vi "Utility - Set 32x32 Picture Values.vi"(8 "error in":errorcluster, 10 "Icon Names":string, 11 "Picture Refnums":refnum<vi>[](array[refnum])) -> (0 "error out":errorcluster)   [LabVIEW 2014]
doc: "::: VI Helpeks :::\nCopyright (c) 2000-2026 Konstantin Shifershteyn. All rights reserved."
panel:
  # "VI Helpeks\nCopyright (c) 2012-2026 Konstantin Shifershteyn"
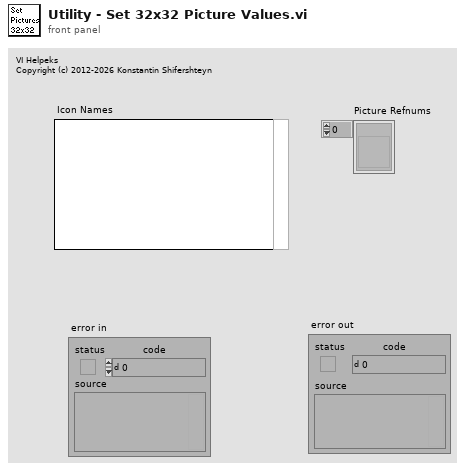
[diagram p1: front panel]
types:
  T1 = typedef "imagedata.ctl" = cluster{"image type":i32, "image depth":i32, "image":u8[], "mask":u8[], "colors":u32[], "Rectangle":cluster{"left":i16, "top":i16, "right":i16, "bottom":i16}}
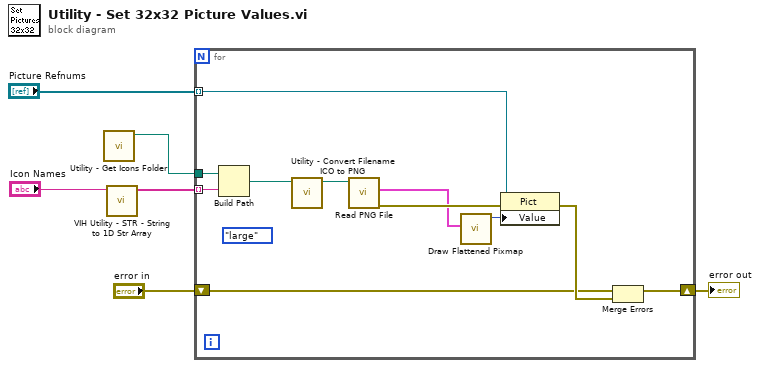
[diagram p0: block diagram]
diagram:
  n1 = call "Utility - Get Icons Folder.vi"() -> ("Icons Folder"=w3:path)  [unwired: 10 in, 1 out]
  n2 = call "VIH Utility - STR - String to 1D Str Array.vi"("String in"="Icon Names") -> ("Array out"=w6:string[])  [unwired: 6 in]
  n3 = for {
    tunnel: w6 -> [w17] mode=indexing
    tunnel: "Picture Refnums" -> [w16] mode=indexing
    tunnel: w3 -> [w12]
    shift-right: [w9] -> w1
    shift-left: "error in" -> [w10]
    (unwired) enum32{"small", "large"}."large" ("Icon type (small)")
    n4 = Build Path(base path=w12, name or relative path=w17) -> (appended path=w8:path)
    n5 = call "Utility - Convert Filename ICO to PNG.vi"("Path"=w8) -> ("Path 2"=w7:path)  [unwired: 10 in]
    n6 = call <vilib>:"Read PNG File.vi"("path to PNG file"=w7) -> ("error out"=w14:errorcluster, "image data"=w13:T1)  [unwired: 8 in, 1 out]
    n7 = call <vilib>:"Draw Flattened Pixmap.vi"("image data"=w13) -> ("new picture"=w15:picture)  [unwired: 8 in]
    n8 = property class="Pict"(reference=w16, error in=w14, "Value"=w15) -> (error out=w11:errorcluster)  [unwired: 1 out]
    n9 = Merge Errors(w10, w11) -> (w9:errorcluster)
  }
  "error out" <- w1
